vi "CAL-Apply ANSI RETSPL Values.vi"(0 "ASTF Mag in":dbl[](array[numeric]), 2 "Speaker":string, 5 "ASTF Phase in":dbl[](array[numeric]), 7 "Frequency in":dbl[](array[numeric]), 11 "error in (no error)":errorcluster) -> (4 "ASTF Mag out":dbl[](array[numeric]), 6 "ASTF Phase out":dbl[](array[numeric]), 8 "Frequency out":dbl[](array[numeric]), 15 "error out":errorcluster)   [LabVIEW 2020]
uses:
  c203f770-9c10-4973-bd8e-152b5d447d6c.vi
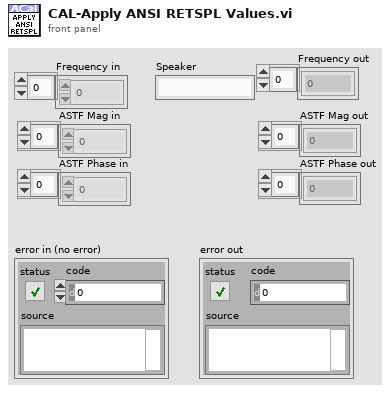
[diagram p1: front panel]
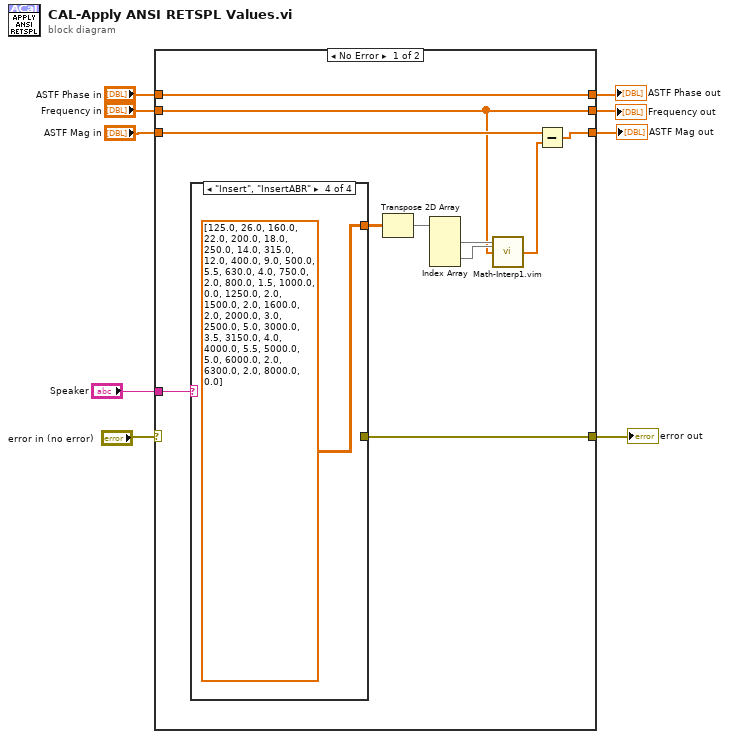
[diagram p0: block diagram]
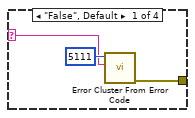
[diagram p2: hidden frame]
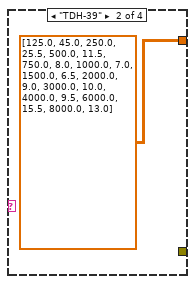
[diagram p3: hidden frame]
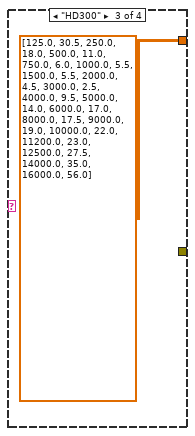
[diagram p4: hidden frame]
diagram:
  n1 = case shown="No Error" "error in (no error)" {
    selector: "error in (no error)" -> [_ w27]
    tunnel: [w16 w27] -> w2
    tunnel: "ASTF Mag in" -> [w20 w28]
    tunnel: "ASTF Phase in" -> [w19 w30]
    tunnel: "Frequency in" -> [w12 w29]
    tunnel: [w11 w28] -> w6
    tunnel: [w19 w30] -> w7
    tunnel: [w12 w29] -> w8
    tunnel: "Speaker" -> [w18 _]
    frame No Error {
      n2 = case shown="\"Insert\", \"InsertABR\"" w18 {
        selector: w18 -> [w22 _ _ _]
        tunnel: [_ dbl[][] [[125.0, 45.0], [250.0, 25.5], [500.0, 11.5], [750.0, 8.0], [1000.0, 7.0], [1500.0, 6.5], [2000.0, 9.0], [3000.0, 10.0], [4000.0, 9.5], [6000.0, 15.5], [8000.0, 13.0]] dbl[][] [[125.0, 30.5], [250.0, 18.0], [500.0, 11.0], [750.0, 6.0], [1000.0, 5.5], [1500.0, 5.5], [2000.0, 4.5], [3000.0, 2.5], [4000.0, 9.5], [5000.0, 14.0], [6000.0, 17.0], [8000.0, 17.5], [9000.0, 19.0], [10000.0, 22.0], [11200.0, 23.0], [12500.0, 27.5], [14000.0, 35.0], [16000.0, 56.0]] dbl[][] [[125.0, 26.0], [160.0, 22.0], [200.0, 18.0], [250.0, 14.0], [315.0, 12.0], [400.0, 9.0], [500.0, 5.5], [630.0, 4.0], [750.0, 2.0], [800.0, 1.5], [1000.0, 0.0], [1250.0, 2.0], [1500.0, 2.0], [1600.0, 2.0], [2000.0, 3.0], [2500.0, 5.0], [3000.0, 3.5], [3150.0, 4.0], [4000.0, 5.5], [5000.0, 5.0], [6000.0, 2.0], [6300.0, 2.0], [8000.0, 0.0]]] -> w17
        tunnel: [w21 _ _ _] -> w16
        frame "False", Default {
          n3 = call <vilib>:"Error Cluster From Error Code.vi"("error message (\"\")"=w22, "error code (0)"=5111) -> ("error out"=w21:errorcluster)  [unwired: 7 in]
        }
        frame "TDH-39" {
        }
        frame "HD300" {
        }
        frame "Insert", "InsertABR" {
        }
      }
      n4 = Transpose 2D Array(2D array=w17) -> (transposed array=w15:dbl[][])
      n5 = Index Array(array=w15) -> (element #1=w14:dbl[], element #2=w13:dbl[])  [unwired: 4 in]
      n6 = call "Math-Interp1.vim"("X"=w14, "Y"=w13, "U"=w12) -> ("V"=w10:dbl[])  [unwired: 12 in]
      n7 = Subtract(x=w20, y=w10) -> (x-y=w11:dbl[])
    }
    frame Error {
    }
  }
  "Frequency out" <- w8
  "ASTF Phase out" <- w7
  "ASTF Mag out" <- w6
  "error out" <- w2
